vi "espectro-de-una-senal-senoidal.vi"() -> ()   [LabVIEW 2019]
uses:
  <vilib>/express/express analysis/Spectral/Block/exnSpectralBlock spectral measurements PSD poly.vi
  <vilib>/express/express analysis/Spectral/Block/exnSpectralBlock spectral measurements PSD DDT.vi
  <vilib>/express/express analysis/Spectral/XNode/ExpressSpectralMeasurementsBlockNode.xnode
panel:
  in  "stop":bool
  in  "Frecuencia":dbl(knob) scale=0.0..500.0
  in  "Amplitud":dbl(slide) scale=1.0..10.0
  out "Potencia espectral":dynamicdata(graph)
  out "Señal original":dynamicdata(graph)
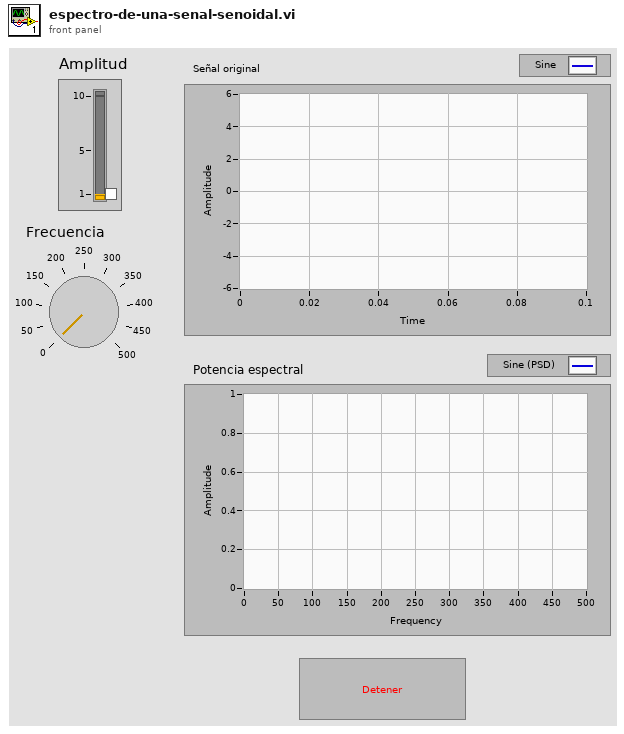
[diagram p1: front panel]
types:
  T1 = cluster{"averaging mode":u16, "weighting mode":u16, "number of averages":u32}
  T2 = cluster{"dB On (F)":bool, "unwrap phase (F)":bool, "convert to degree (F)":bool}
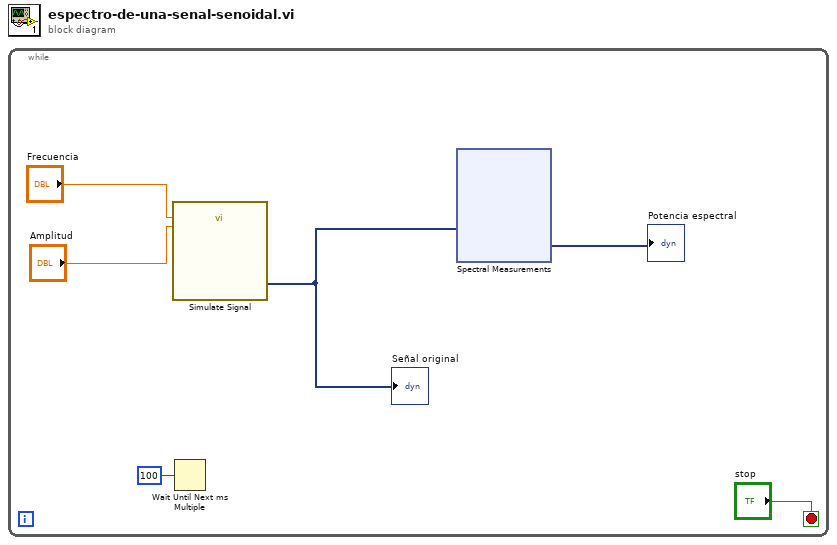
[diagram p0: block diagram]
diagram:
  n1 = while {
    stop <- "stop" stop-if-true
    n2 = call "Simulate Signal"("Frequency"="Frecuencia", "Amplitude"="Amplitud") -> ("Sine"=w5:dynamicdata)  [unwired: 12 in, 1 out]
    "Señal original" <- w5
    n3 = Wait Until Next ms Multiple(millisecond multiple=u32 100) -> ()  [unwired: 1 out]
    n4 = xnode "Spectral Measurements"("Signals"=w5) -> ("PSD"=→"Potencia espectral":dynamicdata)  [unwired: 1 in, 1 out]
  }
